vi "Factorial.vi"() -> ()   [LabVIEW 2026]
panel:
  out "Not Valid Input?":bool
  out "Factorial Result":i64
  in  "Input Number(N)":i64
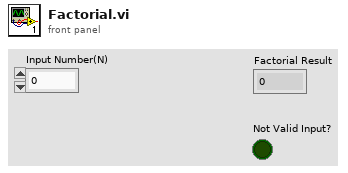
[diagram p1: front panel]
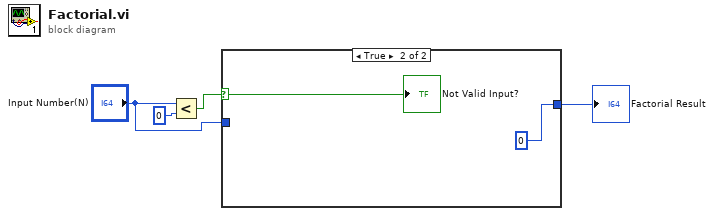
[diagram p0: block diagram]
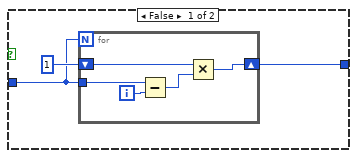
[diagram p2: hidden frame]
diagram:
  n1 = Less?(x="Input Number(N)", y=i64 0) -> (x < y?=w1:bool)
  n2 = case shown="True" w1 {
    selector: w1 -> [_ w13]
    tunnel: "Input Number(N)" -> [w6 _]
    tunnel: [w5 i64 0] -> w2
    frame False {
      n3 = for {
        N: w6 -> [_]
        shift-right: [w8] -> w5
        shift-left: i64 1 -> [w12]
        tunnel: w6 -> [w10]
        i -> [w11]
        n4 = Subtract(x=w10, y=w11) -> (x-y=w9:i64)
        n5 = Multiply(x=w12, y=w9) -> (x*y=w8:i64)
      }
    }
    frame True {
      "Not Valid Input?" <- w13
    }
  }
  "Factorial Result" <- w2
